vi "macro_PIDController_AdvExecute.vi"() -> ()   [LabVIEW 2019, in "Trajectory_Library.lvlib"]
uses:
  Trajectory_Library.lvlib
panel:
  in  "FF-FeedForward":dbl
  in  "SP-SetPoint":dbl
  in  "PV-Measurement":dbl
  out "CO-ControlOutput":dbl
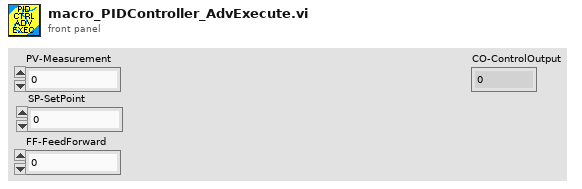
[diagram p1: front panel]
types:
  T1 = typedef "Trajectory_Library.lvlib/PID_ADV_LIMITS.ctl" = cluster{"MaxInput":dbl, "MinInput":dbl, "Continuous":bool, "MaxOutput":dbl, "MinOutput":dbl}
  T2 = typedef "Trajectory_Library.lvlib/PID_ADV_TUNING.ctl" = cluster{"Kf":dbl, "Kp":dbl, "Ki":dbl, "Kd":dbl, "MaximumIntegral":dbl, "MinimumIntegral":dbl, "Filter Derivative":bool, "IntegralZone":dbl}
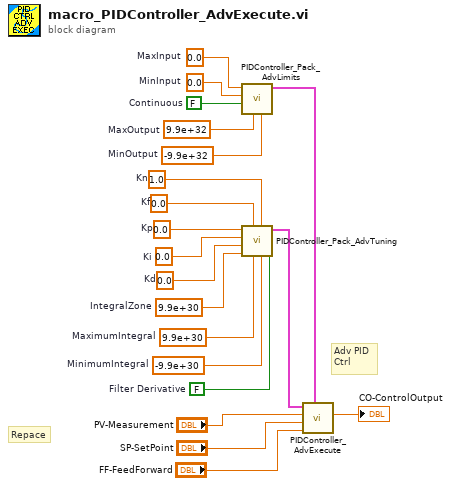
[diagram p0: block diagram]
diagram:
  w5 = 9.9e+30  # IntegralZone
  w6 = 1.0  # Kn
  w7 = 0.0  # Kp
  w8 = 0.0  # Ki
  w9 = 0.0  # Kd
  w10 = 0.0  # Kf
  w11 = 9.9e+30  # MaximumIntegral
  w12 = -9.9e+30  # MinimumIntegral
  w13 = FALSE  # Filter Derivative
  w15 = 0.0  # MinInput
  w16 = FALSE  # Continuous
  w17 = 9.9e+32  # MaxOutput
  w14 = -9.9e+32  # MinOutput
  w18 = 0.0  # MaxInput
  # "Repace"
  # "Adv PID\nCtrl"
  n1 = call "PIDController_Pack_AdvLimits.vi"("MinOutput"=w14, "MaxOutput"=w17, "Continuous"=w16, "MinInput"=w15, "MaxInput"=w18) -> ("Adv PID Limits"=w20:T1)  [unwired: 6 in]
  n2 = call "PIDController_Pack_AdvTuning.vi"("Filter Derivative"=w13, "MinimumIntegral"=w12, "Kn"=w6, "MaximumIntegral"=w11, "Kf"=w10, "IntegralZone"=w5, "Kd"=w9, "Ki"=w8, "Kp"=w7) -> ("Adv PID Tuning"=w19:T2)  [unwired: 2 in]
  n3 = call "PIDController_AdvExecute.vi"("Adv PID Limits"=w20, "FF-FeedForward"="FF-FeedForward", "SP-SetPoint"="SP-SetPoint", "PV-Measurement"="PV-Measurement", "Adv PID Tuning"=w19) -> ("CO-ControlOutput"=→"CO-ControlOutput":dbl)  [unwired: 4 in, 2 out]
